vi "Get Sheet byName.vi"(8 "error IO":errorcluster, 10 "SheetName":string, 11 "ooCalc in":refnum<class "ooCalc.lvclass">) -> (0 "error out":errorcluster, 2 "Sheet":refnum<k24>, 3 "ooCalc out":refnum<class "ooCalc.lvclass">)   [LabVIEW 2009, in "ooCalc.lvclass"]
uses:
  ooCalc.lvclass
  C:/Projets/LAVAG/OpenOfficeRGT/AODL/DLLs/AODL.dll
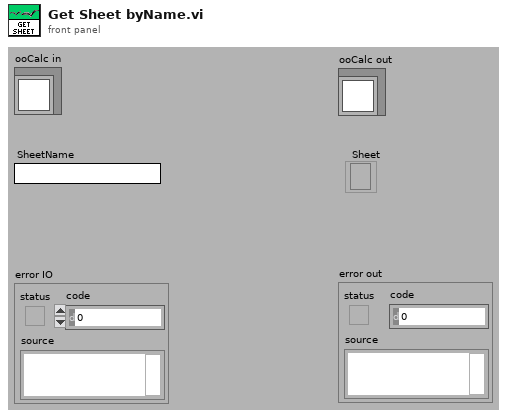
[diagram p1: front panel]
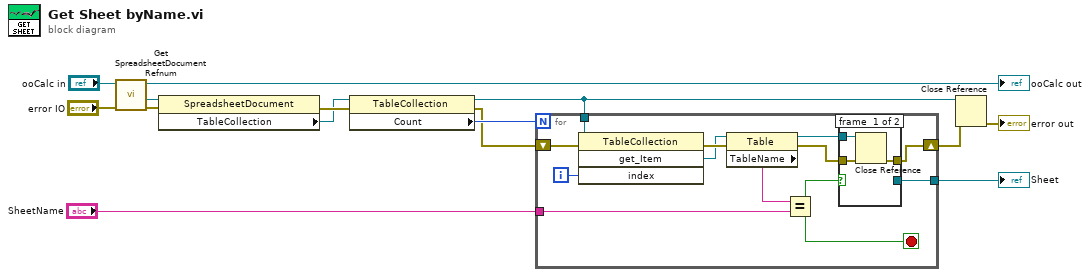
[diagram p0: block diagram]
diagram:
  n1 = call-dynamic "Get SpreadsheetDocument Refnum.vi"("error in (no error)"="error IO", "ooCalc in"="ooCalc in") -> ("error out"=w1:errorcluster, "SpreadsheetDocument"=w5:refnum<k24>, "ooCalc out"=→"ooCalc out":refnum<class "ooCalc.lvclass">)  [unwired: 7 in]
  n2 = property class="SpreadsheetDocument"(reference=w5, error in=w1) -> (error out=w13:errorcluster, "TableCollection"=w12:refnum<k24>)  [unwired: 1 out]
  n3 = property class="TableCollection"(reference=w12, error in=w13) -> (reference out=w10:refnum<k24>, error out=w9:errorcluster, "Count"=w11:i32)
  n4 = for {
    N: w11 -> [_]
    tunnel: w10 -> [w23]
    shift-right: [w21] -> w8
    shift-left: w9 -> [w22]
    tunnel: "SheetName" -> [w18]
    tunnel: [w16] -> w6
    i -> [w26]
    stop <- w15 stop-if-true
    n5 = invoke class="TableCollection" method="get_Item"(reference=w23, error in=w22, "index"=w26) -> (error out=w25:errorcluster, "get_Item"=w19:refnum<k24>)  [unwired: 1 in, 2 out]
    n6 = property class="Table"(reference=w19, error in=w25) -> (reference out=w24:refnum<k24>, error out=w20:errorcluster, "TableName"=w17:string)
    n7 = Equal?(x=w17, y=w18) -> (x = y?=w15:bool)
    n8 = case shown="False" w15 {
      tunnel: w24 -> [w29 w31]
      tunnel: [w28 w30] -> w21
      tunnel: w20 -> [w27 w30]
      tunnel: [_ w31] -> w16
      frame #0 {
        n9 = Close Reference(reference=w29, error in (no error)=w27) -> (error out=w28:errorcluster)
      }
      frame #1 {
      }
    }
  }
  "Sheet" <- w6
  n10 = Close Reference(reference=w10, error in (no error)=w8) -> (error out=→"error out":errorcluster)
